vi "test calc T50 T90 T100.vi"() -> ()   [LabVIEW 2019]
panel:
  out "value":T1
  out "standard error":string
  out "standard output":string
  out "error out 2":errorcluster
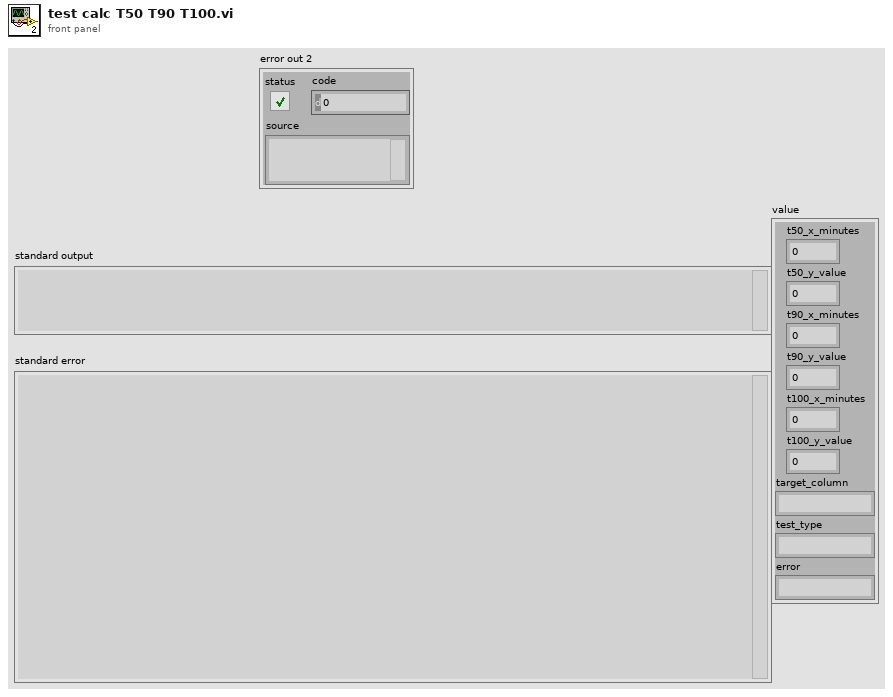
[diagram p1: front panel]
types:
  T1 = cluster{"t50_x_minutes":dbl, "t50_y_value":dbl, "t90_x_minutes":dbl, "t90_y_value":dbl, "t100_x_minutes":dbl, "t100_y_value":dbl, "target_column":string, "test_type":string, "error":string}
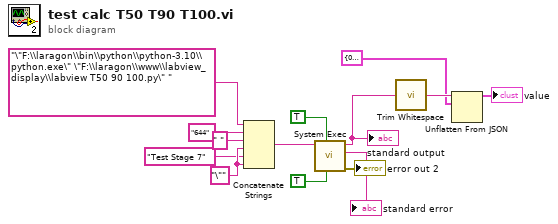
[diagram p0: block diagram]
diagram:
  w8 = "\"" ("string")
  n1 = Concatenate Strings("\"F:\\laragon\\bin\\python\\python-3.10\\python.exe\" \"F:\\laragon\\www\\labview_display\\labview T50 90 100.py\" " ("command line"), "644" ("string"), " " ("string"), w8, "Test Stage 7" ("string"), w8) -> (w7:string)
  n2 = call <vilib>:"System Exec.vi"("run minimized? (F)"=TRUE, "wait until completion? (T)"=TRUE, "command line"=w7) -> ("error out"=→"error out 2":errorcluster, "standard error"=→"standard error":string, "standard output"=w1:string)  [unwired: 5 in, 1 out]
  "standard output" <- w1
  n3 = call <vilib>:"Trim Whitespace.vi"("string"=w1) -> ("trimmed string"=w4:string)  [unwired: 1 in]
  n4 = Unflatten From JSON(JSON string=w4, type and defaults=T1 {"t50_x_minutes"=0.0, "t50_y_value"=0.0, "t90_x_minutes"=0.0, "t90_y_value"=0.0, "t100_x_minutes"=0.0, "t100_y_value"=0.0, "target_column"="", "test_type"="", "error"=""}) -> (value=→"value":T1)  [unwired: 5 in, 1 out]
